vi "Format Wall Time.vi"(4 "Unix ns":i64) -> (7 "String":string)   [LabVIEW 2020, in "VolatusSeqGUI.lvlib" / "Sequencing Control.lvclass"]
uses:
  Sequencing Control.lvclass
  Sequencing Control.lvclass/Sequencing Control.ctl
  lv-vecto/Vecto/Vecto.lvlib
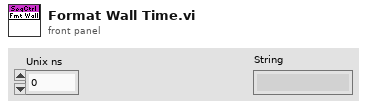
[diagram p1: front panel]
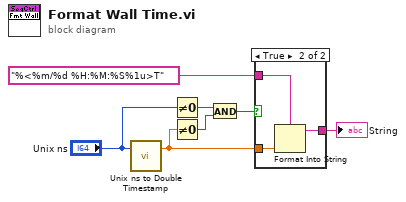
[diagram p0: block diagram]
diagram:
  n1 = call "Unix ns to Double Timestamp.vi"("unix ns"="Unix ns") -> ("Timestamp"=w6:dbl)  [unwired: 2 in]
  n2 = Not Equal To 0?(x="Unix ns") -> (x != 0?=w3:bool)
  n3 = Not Equal To 0?(x=w6) -> (x != 0?=w2:bool)
  n4 = And(x=w3, y=w2) -> (x .and. y?=w1:bool)
  n5 = case shown="True" w1 {
    tunnel: [_ w10] -> w7
    tunnel: w6 -> [_ w9]
    tunnel: "%<%m/%d %H:%M:%S%1u>T" -> [_ w8]
    frame False {
    }
    frame True {
      n6 = Format Into String(format string=w8, w9) -> (resulting string=w10:string)  [unwired: 2 in, 1 out]
    }
  }
  "String" <- w7
